vi "Response Status Code.vi"(10 "has id":bool, 11 "response":string) -> (3 "status code":u16)   [LabVIEW 2020, in "MCP Server.lvlib"]
doc: "HTTP status code for an answer of the request handler: 202 when there is nothing to answer (response is empty and the request has no id, i.e. a notification), otherwise 200. Used by Complete Modern MCP Result.vi."
uses:
  MCP Server.lvlib
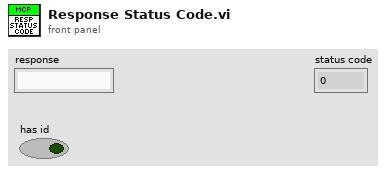
[diagram p1: front panel]
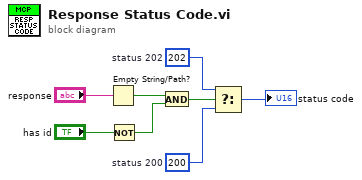
[diagram p0: block diagram]
diagram:
  w4 = u16 200  # status 200
  w3 = u16 202  # status 202
  n1 = Empty String/Path?(string/path="response") -> (empty?=w5:bool)
  n2 = Not(x="has id") -> (.not. x?=w6:bool)
  n3 = And(x=w5, y=w6) -> (x .and. y?=w7:bool)
  n4 = Select(t=w3, s=w7, f=w4) -> (s? t:f=→"status code":u16)
